vi "ingest_csv.vi"(4 "optional":T1, 7 "timestampMetadata":refnum<class "timestampMetadata.lvclass">, 8 "error in":errorcluster, 9 "Target":refnum<class "target.lvclass">, 10 "Source":refnum<class "source.lvclass">, 11 "Nominal Client in":refnum<class "Nominal Client.lvclass">) -> (0 "error out":errorcluster, 1 "datasetFileId":string, 2 "datasetRid":string, 3 "Nominal Client out":refnum<class "Nominal Client.lvclass">)   [LabVIEW 2020, in "Nominal Client.lvclass"]
doc: "Triggers an ingest job, allowing either creating a new dataset or uploading to an existing one. This endpoint is meant to supersede all other ingestion endpoints as their functionality gets migrated to this one."
uses:
  Nominal Client.lvclass
  datasources/target/target.lvclass
  datasources/source/source.lvclass
  timestampMetadata/timestampMetadata.lvclass
  Nominal Client.lvclass/Nominal Client.ctl
  datasources/target/target.lvclass/target.ctl
  4e81ab5e-e540-474e-8302-0a664eb7b944.vi
  da70c7dd-7914-44ef-86ed-2bc4582d2eab.vi
  datasources/target/workspace.set.vi
  trace.payload_received.vi
  error.vi
  trace.payload_sent.vi
  create.authorization_header.vi
  trace.calling_method.vi
  error.vi/859f8e04-e495-489b-b5b4-7ac163f56130.vi
  <vilib>/JDP Science/JDP Science Common Utilities/Trim Whitespace__JDP.vi
  <vilib>/AdvancedString/1D String Array to Delimited String.vi
  api_token.get.vi
  <vilib>/JDP Science/JSONtext/Variant to JSON Text.vi
  <vilib>/JDP Science/JSONtext/support/Format JSON Object.vi
  <vilib>/Utility/libraryn.llb/Get File Extension.vi
  log_file.write.vi
  submodules/reqwest-labview/lv-src/reqwest/post.vi
  <vilib>/JDP Science/JSONtext/Get all Object Items.vi
  <vilib>/Utility/error.llb/Error Cluster From Error Code.vi
  <vilib>/JDP Science/JSONtext/JSON text to Variant.vi
  <vilib>/JDP Science/JSONtext/LVClass Serializer/JSONtext LVClass Serializer.lvclass
  nominal types/properties/properties.lvclass
  nominal types/labels/labels.lvclass
  <vilib>/JDP Science/JSONtext/JSONtext.lvlib
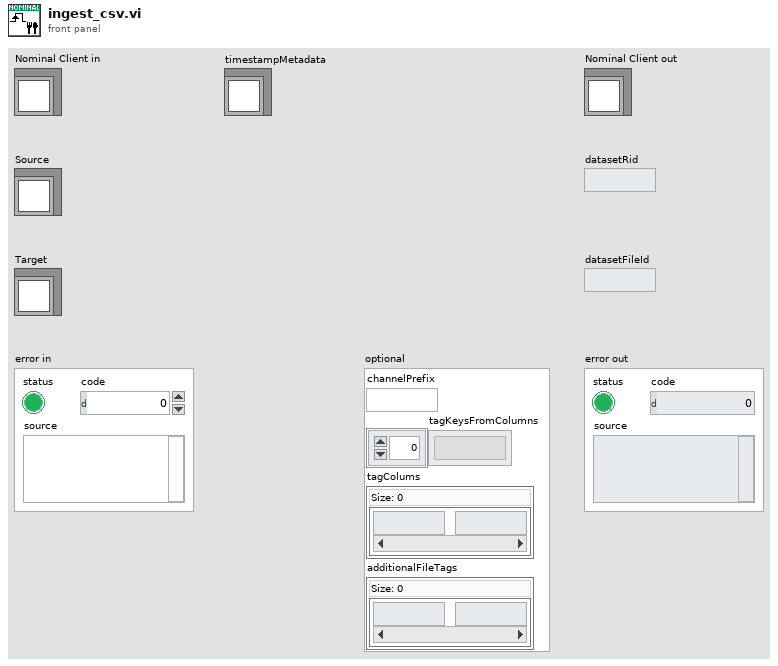
[diagram p1: front panel]
types:
  T1 = cluster{"channelPrefix":string, "tagKeysFromColumns":string[], "tagColums":map{string, string}, "additionalFileTags":map{string, string}}
  T2 = cluster{"type":string, "dataset":cluster{"datasetFileId":string, "datasetRid":string}}
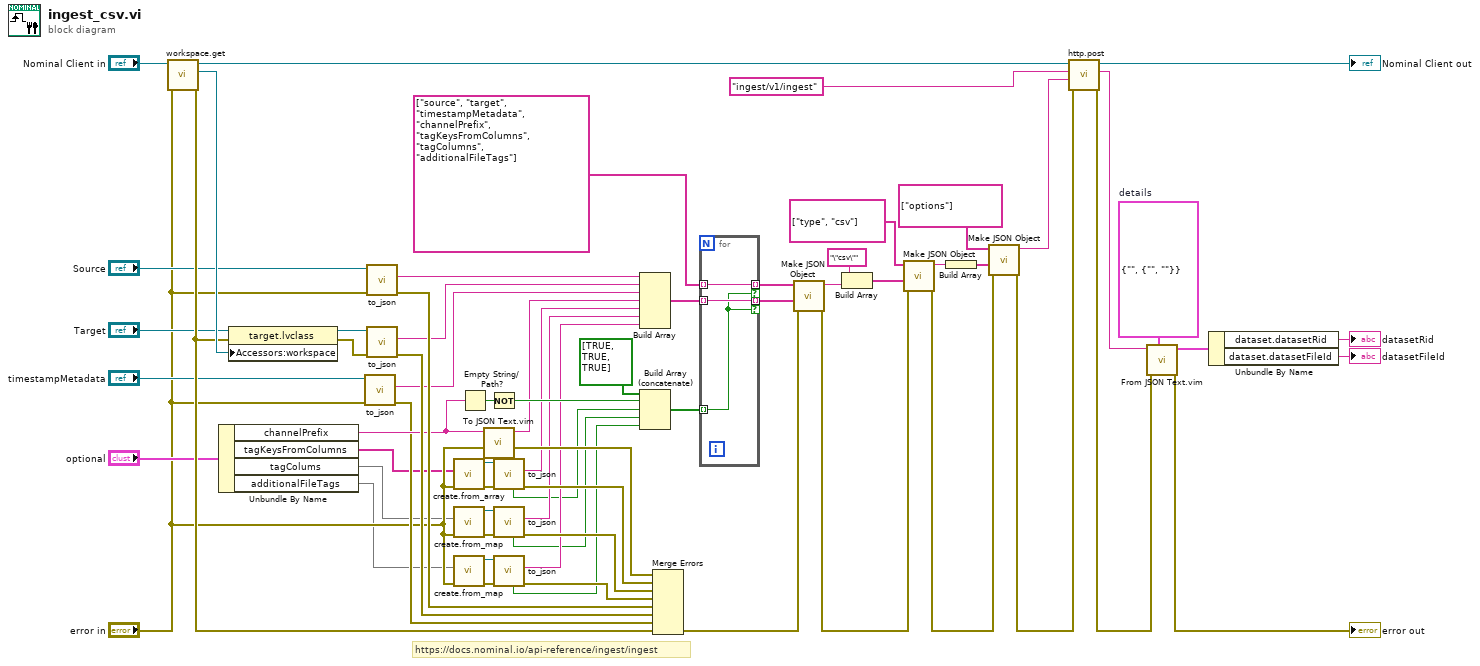
[diagram p0: block diagram]
diagram:
  w23 = T2 {"type"="", "dataset"={"datasetFileId"="", "datasetRid"=""}}  # details
  # "https://docs.nominal.io/api-reference/ingest/ingest"
  n1 = call "workspace.get.vi"("error in"="error in", "Nominal Client in"="Nominal Client in") -> ("error out"=w45:errorcluster, "workspace"=w59:refnum<class "workspace.lvclass">, "Nominal Client out"=w60:refnum<class "Nominal Client.lvclass">)  [unwired: 7 in]
  n2 = Unbundle By Name("optional") -> ("channelPrefix"=w54:string, "tagKeysFromColumns"=w1:string[], "tagColums"=w2:map{string, string}, "additionalFileTags"=w3:map{string, string})
  n3 = property class="target.lvclass"(reference="Target", error in=w45, "Accessors:workspace"=w59) -> (reference out=w62:refnum<class "target.lvclass">, error out=w63:errorcluster)
  n4 = call-dynamic "to_json.vi"("error in"="error in", "timestampMetadata in"="timestampMetadata") -> ("error out"=w44:errorcluster, "json"=w56:string)  [unwired: 6 in, 2 out]
  n5 = call-dynamic "to_json.vi"("error in"="error in", "source in"="Source") -> ("error out"=w65:errorcluster, "json"=w58:string)  [unwired: 6 in, 2 out]
  n6 = call-dynamic "to_json.vi"("error in"=w63, "target in"=w62) -> ("error out"=w64:errorcluster, "json"=w57:string)  [unwired: 6 in, 2 out]
  n7 = call "create.from_array.vi"("error in"="error in", "labels"=w1) -> ("error out"=w5:errorcluster, "labels out"=w6:refnum<class "labels.lvclass">)  [unwired: 8 in]
  n8 = call "create.from_map.vi"("error in"="error in", "properties"=w2) -> ("error out"=w8:errorcluster, "properties out"=w7:refnum<class "properties.lvclass">)  [unwired: 8 in]
  n9 = call "create.from_map.vi"("error in"="error in", "properties"=w3) -> ("error out"=w9:errorcluster, "properties out"=w10:refnum<class "properties.lvclass">)  [unwired: 8 in]
  n10 = Empty String/Path?(string/path=w54) -> (empty?=w55:bool)
  n11 = call "To JSON Text.vim"("error in (no error)"="error in", "Anything"=w54) -> ("error out"=w40:errorcluster, "<JSON>"=w39:string)  [unwired: 8 in]
  n12 = Not(x=w55) -> (.not. x?=w53:bool)
  n13 = call-dynamic "to_json.vi"("error in"=w5, "labels in"=w6) -> ("error out"=w41:errorcluster, "json"=w38:string, "Not Default"=w35:bool)  [unwired: 6 in, 1 out]
  n14 = call-dynamic "to_json.vi"("error in"=w8, "properties in"=w7) -> ("error out"=w42:errorcluster, "json"=w37:string, "Not Default"=w34:bool)  [unwired: 6 in, 1 out]
  n15 = call-dynamic "to_json.vi"("error in"=w9, "properties in"=w10) -> ("error out"=w43:errorcluster, "json"=w36:string, "Not Default"=w33:bool)  [unwired: 6 in, 1 out]
  n16 = Build Array(w58, w57, w56, w39, w38, w37, w36) -> (w51:string[])
  n17 = Build Array (concatenate)(bool[] [TRUE, TRUE, TRUE] ("element"), w53, w35, w34, w33) -> (w47:bool[])
  n18 = Merge Errors(w40, w41, w42, w43, w65, w64, w44, w45) -> (w46:errorcluster)
  n19 = for {
    tunnel: w51 -> [w70] mode=indexing
    tunnel: [w70] -> w50 mode=indexing if=w68
    tunnel: string[] ["source", "target", "timestampMetadata", "channelPrefix", "tagKeysFromColumns", "tagColumns", "additionalFileTags"] ("Item Names") -> [w69] mode=indexing
    tunnel: [w69] -> w48 mode=indexing if=w68
    tunnel: w47 -> [w68] mode=indexing
  }
  n20 = call <vilib>:"Make JSON Object.vi"("error in (no error)"=w46, "JSON Items"=w50, "Item Names"=w48) -> ("error out"=w28:errorcluster, "<JSON>"=w31:string)  [unwired: 7 in]
  n21 = Build Array("\"csv\"" ("JSON"), w31) -> (w30:string[])
  n22 = call <vilib>:"Make JSON Object.vi"("error in (no error)"=w28, "JSON Items"=w30, "Item Names"=string[] ["type", "csv"] ("JSON")) -> ("error out"=w14:errorcluster, "<JSON>"=w16:string)  [unwired: 7 in]
  n23 = Build Array(w16) -> (w17:string[])
  n24 = call <vilib>:"Make JSON Object.vi"("error in (no error)"=w14, "JSON Items"=w17, "Item Names"=string[] ["options"] ("JSON")) -> ("error out"=w13:errorcluster, "<JSON>"=w15:string)  [unwired: 7 in]
  n25 = call "http.post.vi"("error in"=w13, "Request body"=w15, "Path"="ingest/v1/ingest", "Nominal Client in"=w60) -> ("error out"=w20:errorcluster, "Response"=w21:string, "Nominal Client out"=→"Nominal Client out":refnum<class "Nominal Client.lvclass">)  [unwired: 5 in]
  n26 = call "From JSON Text.vim"("Data Type and Default Value"=w23, "error in (no error)"=w20, "JSON"=w21) -> ("error out"=→"error out":errorcluster, "Data out"=w22:T2)  [unwired: 7 in]
  n27 = Unbundle By Name(w22) -> ("dataset.datasetRid"=→"datasetRid":string, "dataset.datasetFileId"=→"datasetFileId":string)
